vi "[ex ce] History Speed (VM & DBL scalar).vi"() -> ()   [LabVIEW 2021]
doc: "<B>Run speed example</B>\n\nThe VI demonstrates how a variable history affects execution speed.\n\n::: CalcExpress Toolkit :::\nCopyright (c) 2000-2026 Konstantin Shifershteyn. All rights reserved."
panel:
  out "Historic values":dbl[](array[numeric]) format="%#_9g"
  in  "reverse order":bool=TRUE caption="Read history in reversed order"
  in  "number of iterations":i32=100000
  out "read history, ms":u32
  out "speed ratio":dbl format="%.2f"
  out "with history, ms":u32
  out "without history, ms":u32
  in  "history length":i32=10000
  # "*) history length has big sense for memory use but it does not influence a lot on CPU use."
  # "execution time"
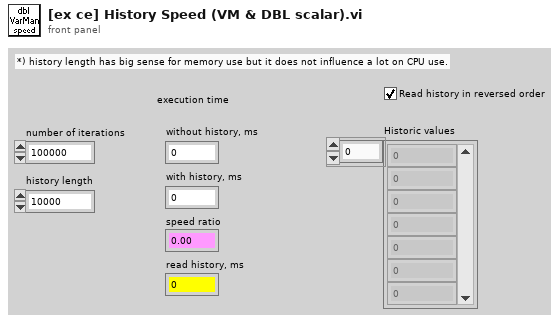
[diagram p1: front panel]
types:
  T1 = enum16{"create", "destroy", "set value", "get value"}
  T2 = enum32{"nop", "create", "destroy", "reset", "get info", "config"}
  T3 = typedef "VarMan Variable Context Handle.ctl" = i32
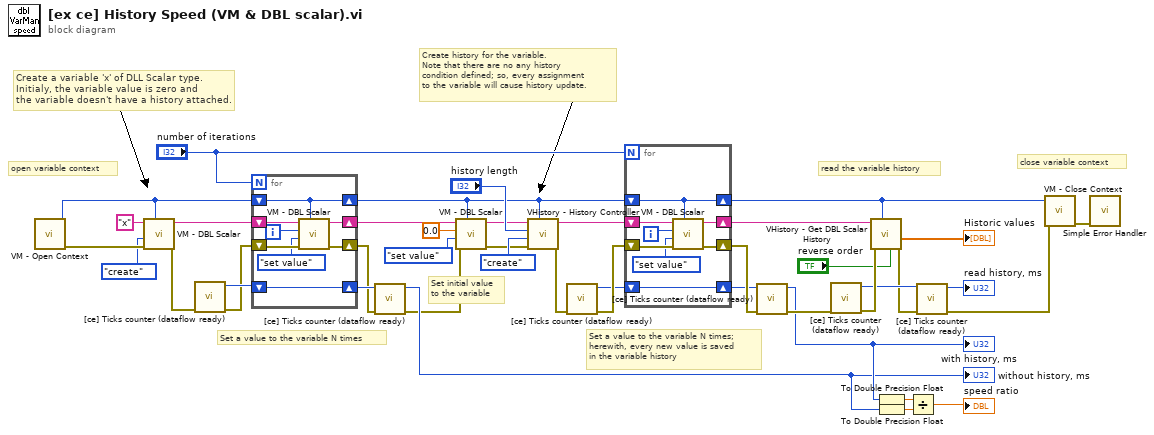
[diagram p0: block diagram]
diagram:
  # "Set initial value\nto the variable"
  # "Create a variable 'x' of DLL Scalar type.\nInitialy, the variable value is zero and\nthe variable doesn't have a history attached."
  # "Create history for the variable.\nNote that there are no any history\ncondition defined; so, every assignment\nto the variable will cause history update."
  # "close variable context"
  # "Set a value to the variable N times;\nherewith, every new value is saved\nin the variable history"
  # "Set a value to the variable N times"
  # "open variable context"
  # "read the variable history"
  n1 = call "VM - Open Context.vi"() -> ("error out"=w42:errorcluster, "VC Handle out"=w25:T3)  [unwired: 9 in, 1 out]
  n2 = call "VM - DBL Scalar.vi"("VC Handle"=w25, "error in"=w42, "cmd"=T1."create", "name_spec"="x" ("name")) -> ("error out"=w26:errorcluster, "dup name_spec"=w27:string)  [unwired: 2 in, 4 out]
  n3 = call "[ce] Ticks counter (dataflow ready).vi"("error in"=w26) -> ("error out"=w38:errorcluster, "ticks (current-input)"=w39:u32)  [unwired: 4 in, 3 out]
  n4 = for {
    N: "number of iterations" -> [_]
    shift-right: [w47] -> w4
    shift-left: w25 -> [w47]
    shift-right: [w49] -> w30
    shift-left: w38 -> [w46]
    shift-right: [w50] -> w5
    shift-left: w27 -> [w48]
    shift-right: [w43] -> w37
    shift-left: w39 -> [w43]
    i -> [w45]
    n5 = call "VM - DBL Scalar.vi"("VC Handle"=w47, "error in"=w46, "cmd"=T1."set value", "value in"=w45, "name_spec"=w48) -> ("error out"=w49:errorcluster, "dup name_spec"=w50:string)  [unwired: 1 in, 4 out]
  }
  n6 = call "[ce] Ticks counter (dataflow ready).vi"("error in"=w30, "ticks in"=w37) -> ("error out"=w1:errorcluster, "ticks (current-input)"=w13:u32)  [unwired: 3 in, 3 out]
  "without history, ms" <- w13
  n7 = call "VM - DBL Scalar.vi"("VC Handle"=w4, "error in"=w1, "cmd"=T1."set value", "value in"=0.0, "name_spec"=w5) -> ("error out"=w2:errorcluster, "dup name_spec"=w3:string)  [unwired: 1 in, 4 out]
  n8 = call "VHistory - History Controller.vi"("VC Handle"=w4, "error in"=w2, "cmd (nop:default)"=T2."create", "history length"="history length", "name_spec"=w3) -> ("error out"=w29:errorcluster, "dup name_spec"=w28:string)  [unwired: 3 in, 2 out]
  n9 = call "[ce] Ticks counter (dataflow ready).vi"("error in"=w29) -> ("error out"=w32:errorcluster, "ticks (current-input)"=w31:u32)  [unwired: 4 in, 3 out]
  n10 = for {
    N: "number of iterations" -> [_]
    shift-right: [w55] -> w19
    shift-left: w4 -> [w55]
    shift-right: [w57] -> w34
    shift-left: w32 -> [w54]
    shift-right: [w58] -> w24
    shift-left: w28 -> [w56]
    shift-right: [w51] -> w33
    shift-left: w31 -> [w51]
    i -> [w53]
    n11 = call "VM - DBL Scalar.vi"("VC Handle"=w55, "error in"=w54, "cmd"=T1."set value", "value in"=w53, "name_spec"=w56) -> ("error out"=w57:errorcluster, "dup name_spec"=w58:string)  [unwired: 1 in, 4 out]
  }
  n12 = call "[ce] Ticks counter (dataflow ready).vi"("error in"=w34, "ticks in"=w33) -> ("error out"=w23:errorcluster, "ticks (current-input)"=w14:u32)  [unwired: 3 in, 3 out]
  "with history, ms" <- w14
  n13 = call "[ce] Ticks counter (dataflow ready).vi"("error in"=w23) -> ("error out"=w22:errorcluster, "ticks (current-input)"=w21:u32)  [unwired: 4 in, 3 out]
  n14 = call "VHistory - Get DBL Scalar History.vi"("reverse order (T)"="reverse order", "VC Handle"=w19, "error in"=w22, "name_spec"=w24) -> ("error out"=w20:errorcluster, "history"=→"Historic values":dbl[])  [unwired: 3 in, 3 out]
  n15 = To Double Precision Float(number=w14) -> (double precision float=w10:dbl)
  n16 = To Double Precision Float(number=w13) -> (double precision float=w9:dbl)
  n17 = Divide(x=w10, y=w9) -> (x/y=→"speed ratio":dbl)
  n18 = call "[ce] Ticks counter (dataflow ready).vi"("error in"=w20, "ticks in"=w21) -> ("error out"=w18:errorcluster, "ticks (current-input)"=→"read history, ms":u32)  [unwired: 3 in, 3 out]
  n19 = call "VM - Close Context.vi"("error in"=w18, "VC Handle"=w19) -> ("error out"=w17:errorcluster)  [unwired: 8 in, 1 out]
  n20 = call <vilib>:"Simple Error Handler.vi"("error in (no error)"=w17) -> ()  [unwired: 4 in, 5 out]
